vi "calculator.vi"() -> ()   [LabVIEW 2021]
panel:
  out "sum":dbl
  out "difference":dbl
  out "quotient":dbl
  out "product":dbl
  in  "Numeric 2":dbl
  in  "Numeric":dbl
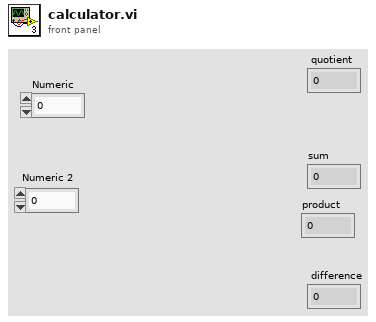
[diagram p1: front panel]
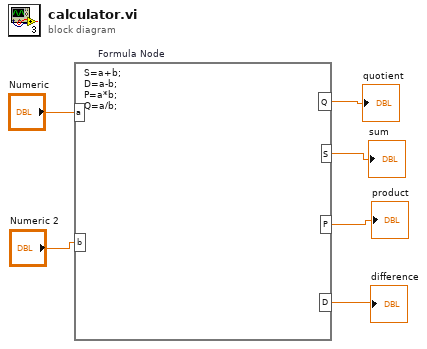
[diagram p0: block diagram]
diagram:
  n1 = formula code="S=a+b;\nD=a-b;\nP=a*b;\nQ=a/b;"("a"="Numeric", "b"="Numeric 2") -> ("Q"=→"quotient":dbl, "S"=→"sum":dbl, "P"=→"product":dbl, "D"=→"difference":dbl)
